vi "VIA Minify all VIs.vi"(11 "VIA in":string) -> (2 "Bytes Removed":i32, 3 "VIA out":string)   [LabVIEW 2020, in "PicoG-Core.lvlib"]
uses:
  PicoG-Core/PicoG-Core.lvlib
  <vilib>/regexp/Match Regular Expression.xnode
panel:
  out "VI types":string[](array[string])
  out "VI Content":string[](array[string])
  out "VI names":string[](array[string])
  out "Number of VIs Processed":i32
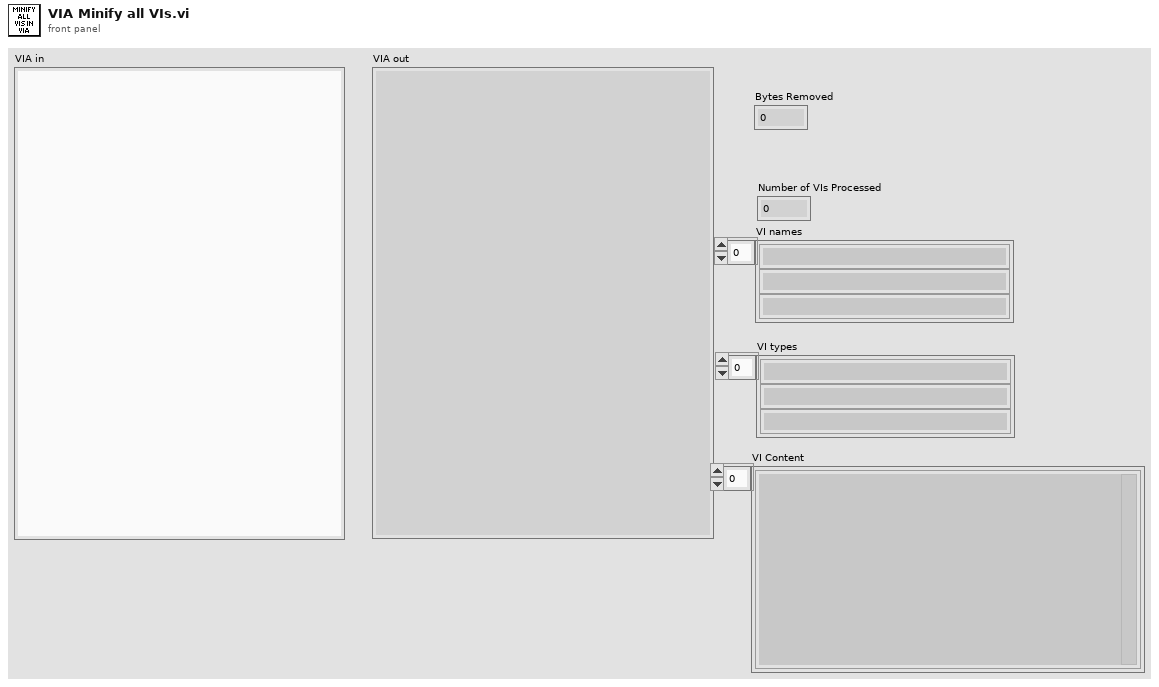
[diagram p1: front panel]
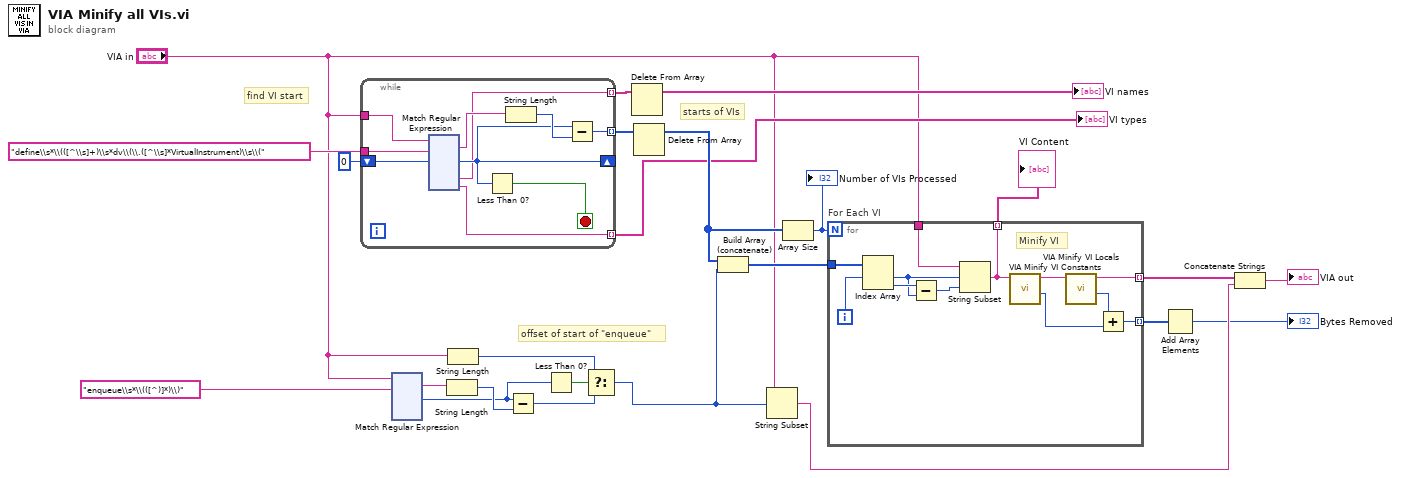
[diagram p0: block diagram]
diagram:
  # "starts of VIs"
  # "offset of start of \"enqueue\""
  # "find VI start"
  n1 = while {
    tunnel: "VIA in" -> [w34]
    tunnel: "define\\s*\\(([^\\s]+)\\s*dv\\(\\.([^\\s]*VirtualInstrument)\\s\\(" ("regular expression") -> [w33]
    shift-right: [w28] -> _
    shift-left: 0 ("offset (0)") -> [w32]
    tunnel: [w29] -> w19 mode=indexing
    tunnel: [w26] -> w10 mode=indexing
    tunnel: [w25] -> w7 mode=indexing
    stop <- w27 stop-if-true
    n2 = xnode "Match Regular Expression"("input string"=w34, "regular expression"=w33, "offset (0)"=w32) -> ("whole match"=w30:string, "offset past match"=w28:i32, "submatch 1"=w26:string, "submatch 2"=w25:string)  [unwired: 3 in, 3 out]
    n3 = Less Than 0?(x=w28) -> (x < 0?=w27:bool)
    n4 = String Length(string=w30) -> (length=w31:i32)
    n5 = Subtract(x=w28, y=w31) -> (x-y=w29:i32)
  }
  "VI types" <- w7
  n6 = xnode "Match Regular Expression"("input string"="VIA in", "regular expression"="enqueue\\s*\\(([^)]*)\\)") -> ("whole match"=w23:string, "offset past match"=w6:i32)  [unwired: 4 in, 4 out]
  n7 = String Length(string=w23) -> (length=w22:i32)
  n8 = String Length(string="VIA in") -> (length=w3:i32)
  n9 = Subtract(x=w6, y=w22) -> (x-y=w2:i32)
  n10 = Less Than 0?(x=w6) -> (x < 0?=w5:bool)
  n11 = Select(t=w3, s=w5, f=w2) -> (s? t:f=w1:i32)
  n12 = Delete From Array(array=w10) -> (array with subset deleted=→"VI names":string[])  [unwired: 2 in, 1 out]
  n13 = Delete From Array(array=w19) -> (array with subset deleted=w16:i32[])  [unwired: 2 in, 1 out]
  n14 = Build Array (concatenate)(w16, w1) -> (w18:i32[])
  n15 = String Subset(string="VIA in", offset (0)=w1) -> (substring=w13:string)  [unwired: 1 in]
  n16 = Array Size(array=w16) -> (size(s)=w17:i32)
  "Number of VIs Processed" <- w17
  n17 = for "For Each VI" {
    N: w17 -> [_]
    tunnel: w18 -> [w163]
    tunnel: "VIA in" -> [w158]
    tunnel: [w154] -> w15 mode=indexing
    tunnel: [w153] -> w14 mode=indexing
    tunnel: [w152] -> w8 mode=indexing
    i -> [w162]
    # "Minify VI"
    n18 = Index Array(array=w163, index #1=w162) -> (element #1=w159:i32, element #2=w161:i32)  [unwired: 1 in]
    n19 = Subtract(x=w161, y=w159) -> (x-y=w160:i32)
    n20 = String Subset(string=w158, offset (0)=w159, length (rest)=w160) -> (substring=w152:string)
    n21 = call "VIA Minify VI Constants.vi"("VIA in"=w152) -> ("Bytes Removes"=w155:i32, "VIA out"=w157:string)  [unwired: 9 in]
    n22 = call "VIA Minify VI Locals.vi"("VIA in"=w157) -> ("Bytes Removes"=w156:i32, "VIA out"=w153:string)  [unwired: 8 in, 1 out]
    n23 = Add(x=w156, y=w155) -> (x+y=w154:i32)
  }
  "VI Content" <- w8
  n24 = Add Array Elements(numeric array=w15) -> (sum=→"Bytes Removed":i32)
  n25 = Concatenate Strings(w14, w13) -> (→"VIA out":string)
